vi "get_roll.vi"(8 "error in (no error)":errorcluster, 11 "ESP32 TRNG":refnum<visa-resource-name>) -> (0 "error out":errorcluster, 1 "from ESP32?":bool, 2 "roll":i32, 3 "ESP32 TRNG":refnum<visa-resource-name>)   [LabVIEW 2026]
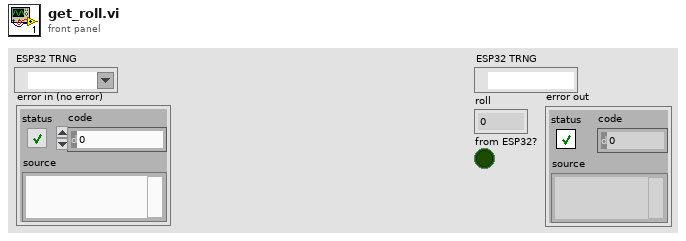
[diagram p1: front panel]
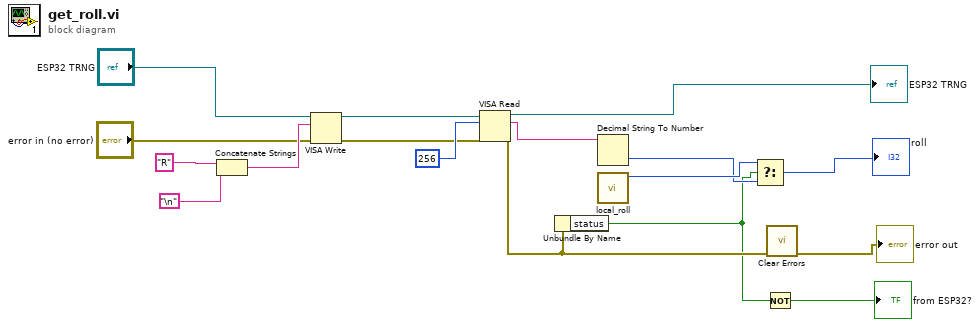
[diagram p0: block diagram]
diagram:
  n1 = Concatenate Strings "Concatenate Strings"("R" ("string"), "\n") -> (w15:string)
  n2 = VISA Write(VISA resource name="ESP32 TRNG", write buffer=w15, error in (no error)="error in (no error)") -> (VISA resource name out=w12:refnum<visa-resource-name>, error out=w10:errorcluster)  [unwired: 1 out]
  n3 = VISA Read(VISA resource name=w12, byte count=u32 256, error in (no error)=w10) -> (VISA resource name out=→"ESP32 TRNG":refnum<visa-resource-name>, read buffer=w9:string, error out=w7:errorcluster)  [unwired: 1 out]
  n4 = Unbundle By Name(w7) -> ("status"=w3:bool)
  n5 = Decimal String To Number(string=w9) -> (number=w5:i32)  [unwired: 2 in, 1 out]
  n6 = call "local_roll.vi"() -> ("number"=w6:i32)  [unwired: 11 in]
  n7 = Select(t=w6, s=w3, f=w5) -> (s? t:f=→"roll":i32)
  n8 = Not(x=w3) -> (.not. x?=→"from ESP32?":bool)
  n9 = call <vilib>:"Clear Errors.vi"("error in (no error)"=w7) -> ("error out"=→"error out":errorcluster)  [unwired: 5 in, 1 out]
